vi "GOOP_CheckClassState.vi"(6 "ClassFileMayBeReadOnly(False)":bool, 8 "error in":errorcluster, 11 "Library Refnum":refnum<vi>) -> (0 "error out":errorcluster)   [LabVIEW 2020]
uses:
  GOOP_ErrorCodes.ctl
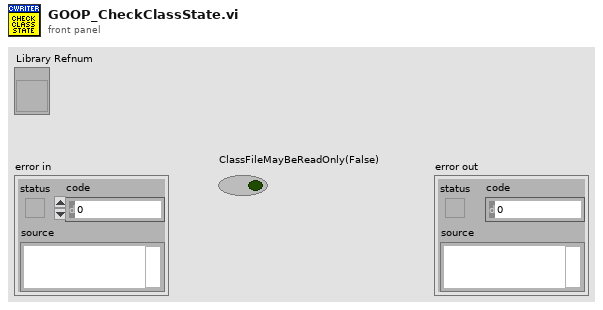
[diagram p1: front panel]
types:
  T1 = typedef "GOOP_ErrorCodes.ctl" = enum16{"LicenseFileMissing", "LicenseFileNotCorrect", "NoProductAccessGranted", "AgreementNoAccepted", "NoValidProviderFound", "LicenseExpired", "LanguageUndefined", "LanguageFileMissing", "LanguageFileChecksumError", "DublicateLanguageTranslation", "LanguageStringIDNotFound", "CommunityLimitReached", "ClassFileLocked", "ClassFileReadOnly", "ProjectNotValid"}
  T2 = enum32{"invalid lock state", "Not Locked", "Locked (No Password)", "Password-protected"}
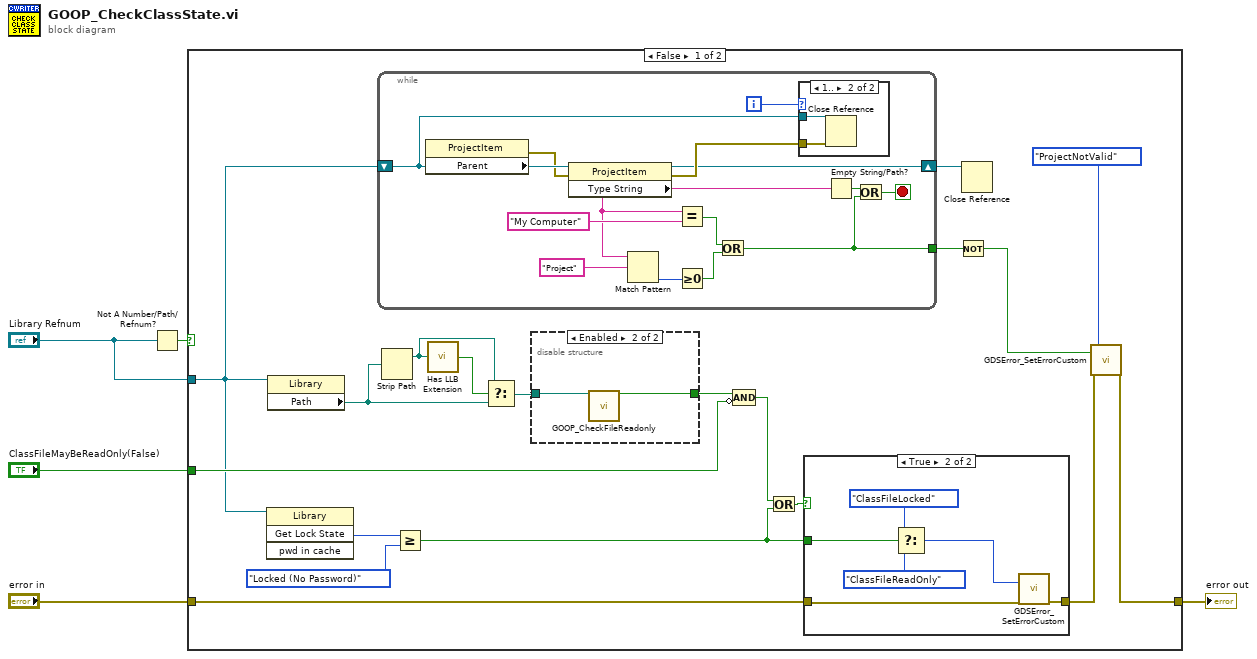
[diagram p0: block diagram]
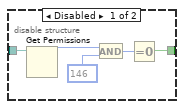
[diagram p2: hidden frame]
diagram:
  n1 = Not A Number/Path/Refnum?(number/path/refnum="Library Refnum") -> (NaN/Path/Refnum?=w4:bool)
  n2 = case shown="False" w4 {
    tunnel: "Library Refnum" -> [w6 _]
    tunnel: "error in" -> [w21 w56]
    tunnel: [w13 w56] -> w3
    tunnel: "ClassFileMayBeReadOnly(False)" -> [w10 _]
    frame False {
      n3 = invoke class="Library" method="Get Lock State"(reference=w6) -> ("Get Lock State"=w24:T2)  [unwired: 3 in, 3 out]
      n4 = property class="Library"(reference=w6) -> ("Path"=w17:path)  [unwired: 1 in, 2 out]
      n5 = while {
        shift-right: [w42] -> w8
        shift-left: w6 -> [w39]
        tunnel: [w32] -> w9
        i -> [w38]
        stop <- w41 stop-if-true
        n6 = property class="ProjectItem"(reference=w39) -> (error out=w44:errorcluster, "Parent"=w46:refnum<vi>)  [unwired: 1 in, 1 out]
        n7 = property class="ProjectItem"(reference=w46, error in=w44) -> (reference out=w42:refnum<vi>, error out=w43:errorcluster, "Type String"=w37:string)
        n8 = Match Pattern(string=w37, regular expression="Project") -> (offset past match=w35:i32)  [unwired: 1 in, 3 out]
        n9 = Equal?(x=w37, y="My Computer") -> (x = y?=w33:bool)
        n10 = Greater Or Equal To 0?(x=w35) -> (x >= 0?=w34:bool)
        n11 = Or(x=w33, y=w34) -> (x .or. y?=w32:bool)
        n12 = case shown="1.." w38 {
          tunnel: w43 -> [_ w48]
          tunnel: w39 -> [_ w47]
          frame 0, Default {
          }
          frame 1.. {
            n13 = Close Reference(reference=w47, error in (no error)=w48) -> ()  [unwired: 1 out]
          }
        }
        n14 = Empty String/Path?(string/path=w37) -> (empty?=w45:bool)
        n15 = Or(x=w45, y=w32) -> (x .or. y?=w41:bool)
      }
      n16 = Strip Path(path=w17) -> (stripped path=w18:path)  [unwired: 1 out]
      n17 = Greater Or Equal?(x=w24, y=T2."Locked (No Password)" ("Lock State:Get")) -> (x >= y?=w20:bool)
      n18 = call <vilib>:"Has LLB Extension.vi"("path"=w18) -> ("path to VI library?"=w19:bool)
      n19 = Select(t=w18, s=w19, f=w17) -> (s? t:f=w16:path)
      n20 = disable-structure shown="Enabled" {
        disable-tunnel: w16 -> [w26 w31]
        disable-tunnel: [w25 w30] -> w12
        frame Disabled {
          n21 = Get Permissions(11:w26) -> (5:w29:i16)  [unwired: 1 in, 4 out]
          n22 = And(x=w29, y=i16 146) -> (x .and. y?=w27:i16)
          n23 = Equal To 0?(x=w27) -> (x = 0?=w25:bool)
        }
        frame Enabled {
          n24 = call "GOOP_CheckFileReadonly.vi"("FilePath"=w31) -> ("IsReadOnly"=w30:bool)  [unwired: 13 in, 1 out]
        }
      }
      n25 = Compound Arithmetic op=AND(w12, invert w10) -> (w11:bool)
      n26 = Or(x=w11, y=w20) -> (x .or. y?=w22:bool)
      n27 = case shown="True" w22 {
        tunnel: w21 -> [w49 w50]
        tunnel: [w49 w55] -> w14
        tunnel: w20 -> [_ w54]
        frame False {
        }
        frame True {
          n28 = Select(t=GOOP_ErrorCodes."ClassFileLocked" ("ErrorCodes"), s=w54, f=GOOP_ErrorCodes."ClassFileReadOnly" ("ErrorCodes")) -> (s? t:f=w51:T1)
          n29 = call "GDSError_SetErrorCustom.vi"("error in (no error)"=w50, "UserDefinedCodes(+5000)"=w51) -> ("error out"=w55:errorcluster)  [unwired: 17 in]
        }
      }
      n30 = Not(x=w9) -> (.not. x?=w7:bool)
      n31 = Close Reference(reference=w8) -> ()  [unwired: 1 in, 1 out]
      n32 = call "GDSError_SetErrorCustom.vi"("status"=w7, "error in (no error)"=w14, "UserDefinedCodes(+5000)"=GOOP_ErrorCodes."ProjectNotValid" ("ErrorCodes")) -> ("error out"=w13:errorcluster)  [unwired: 16 in]
    }
    frame True {
    }
  }
  "error out" <- w3
